vi "OwnOop20261013_SetBooleanConstant.vi"() -> ()   [LabVIEW 2024]
panel:
  out "error out":errorcluster caption="错误输出"
  in  "value":variant
  in  "constant_id":refnum<vi>
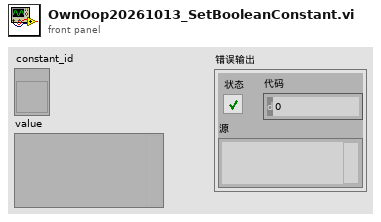
[diagram p1: front panel]
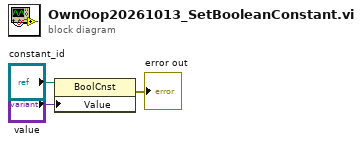
[diagram p0: block diagram]
diagram:
  n1 = property class="BoolCnst"(reference="constant_id", "Value"="value") -> (error out=→"error out":errorcluster)  [unwired: 1 in, 1 out]
